vi "factorial using for loop.vi"() -> ()   [LabVIEW 2021]
panel:
  out "y":i32
  in  "Numeric 2":i32
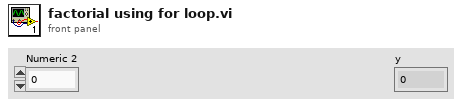
[diagram p1: front panel]
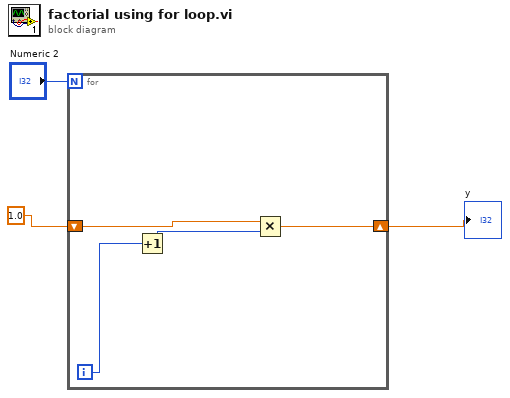
[diagram p0: block diagram]
diagram:
  n1 = for {
    N: "Numeric 2" -> [_]
    shift-right: [w4] -> w1
    shift-left: 1.0 ("x") -> [w6]
    i -> [w5]
    n2 = Increment(x=w5) -> (x+1=w7:i32)
    n3 = Multiply(x=w6, y=w7) -> (x*y=w4:dbl)
  }
  "y" <- w1
